vi "Create Single AO.vi"(7 "section":string, 8 "error in (no error)":errorcluster, 9 "AO_Channel":string(combo)="AO_Channel", 10 "Modbus_Master.lvclass":refnum<class "Modbus_Master.lvclass">, 11 "Config File In":path) -> (0 "error out":errorcluster, 2 "AnalogOutput.lvclass":refnum<class "AnalogOutput.lvclass">, 3 "Config File Out":path)   [LabVIEW 2021]
uses:
  AnalogOutput/AnalogOutput.lvclass
  Modbus_Master/Modbus_Master.lvclass
  Modbus_AO/Modbus_AO.lvclass
  C:/Users/lincoln.lucio/Documents/Lincoln/Documentos Pessoais/meus docs/Projetos pessoais/Projeto Sciranda/projeto_versioned/sciranda/AnalogOutput/AnalogOutput.lvclass
  Modbus_AO/Modbus_AO.lvclass/Modbus_AO.ctl
  DAQNavi_AO.lvclass/DAQNavi_AO.lvclass
  DAQNavi_AO.lvclass/DAQNavi_AO.lvclass/DAQNavi_AO.ctl
  Modbus_AO/Accessor VIs/Write Modbus_Master.lvclass.vi
  Modbus_AO/Accessor VIs/Write Register Address.vi
  Modbus_AO/Accessor VIs/Write Is Signed (I16)_.vi
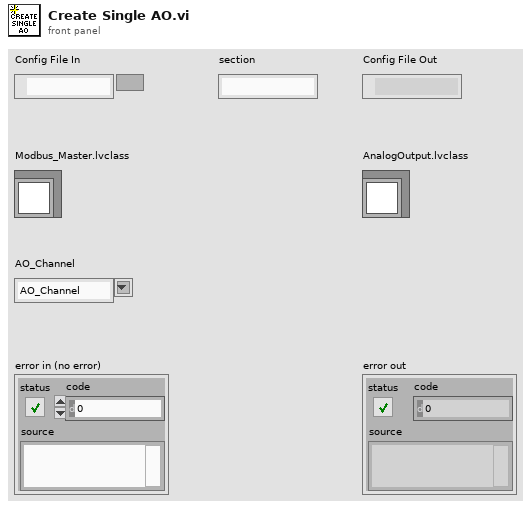
[diagram p1: front panel]
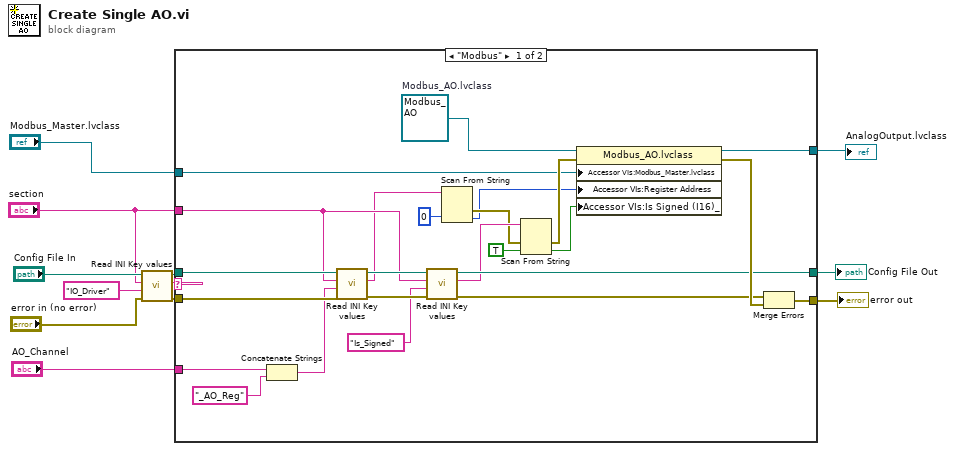
[diagram p0: block diagram]
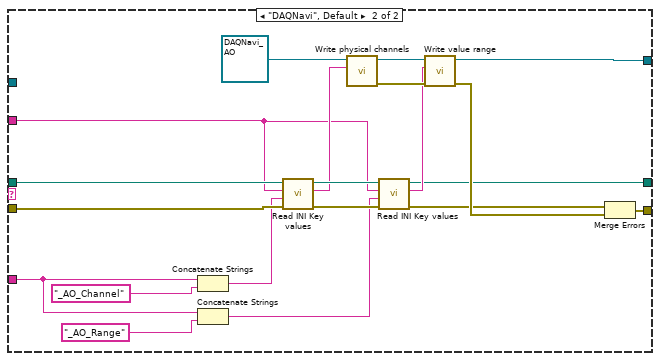
[diagram p2: hidden frame]
diagram:
  n1 = call "Read INI Key values.vi"("error in (no error)"="error in (no error)", "key"="IO_Driver", "section"="section", "Path In"="Config File In") -> ("error out"=w5:errorcluster, "value"=w9:string, "Path Out"=w7:path)  [unwired: 5 in]
  n2 = case shown="\"Modbus\"" w9 {
    tunnel: "AO_Channel" -> [w16 w40]
    tunnel: w7 -> [w32 w49]
    tunnel: w5 -> [w31 w48]
    tunnel: "section" -> [w28 w47]
    tunnel: [w25 w44] -> w11
    tunnel: [w34 w43] -> w10
    tunnel: [w35 w42] -> w3
    tunnel: "Modbus_Master.lvclass" -> [w13 _]
    frame "Modbus" {
      w36 = refnum<class "Modbus_AO.lvclass"> refnum  # Modbus_AO.lvclass
      n3 = Concatenate Strings(w16, "_AO_Reg" ("key")) -> (w14:string)
      n4 = call "Read INI Key values.vi"("error in (no error)"=w31, "key"=w14, "section"=w28, "Path In"=w32) -> ("error out"=w29:errorcluster, "value"=w17:string, "Path Out"=w30:path)  [unwired: 5 in]
      n5 = call "Read INI Key values.vi"("error in (no error)"=w29, "key"="Is_Signed", "section"=w28, "Path In"=w30) -> ("error out"=w26:errorcluster, "value"=w23:string, "Path Out"=w25:path)  [unwired: 5 in]
      n6 = Scan From String(input string=w17, default 1=u16 0 ("Register Address")) -> (error out=w19:errorcluster, output 1=w18:u16)  [unwired: 3 in, 2 out]
      n7 = Scan From String(input string=w23, error in=w19, default 1=TRUE ("Is Signed (I16)_")) -> (error out=w21:errorcluster, output 1=w22:bool)  [unwired: 2 in, 2 out]
      n8 = property class="Modbus_AO.lvclass"(reference=w36, error in=w21, "Accessor VIs:Modbus_Master.lvclass"=w13, "Accessor VIs:Register Address"=w18, "Accessor VIs:Is Signed (I16)_"=w22) -> (reference out=w35:refnum<class "Modbus_AO.lvclass">, error out=w33:errorcluster)
      n9 = Merge Errors(w26, w33) -> (w34:errorcluster)
    }
    frame "DAQNavi", Default {
      n10 = Concatenate Strings(w40, "_AO_Channel" ("string")) -> (w41:string)
      n11 = Concatenate Strings(w40, "_AO_Range" ("string")) -> (w37:string)
      n12 = call "Read INI Key values.vi"("error in (no error)"=w48, "key"=w41, "section"=w47, "Path In"=w49) -> ("error out"=w55:errorcluster, "value"=w54:string, "Path Out"=w56:path)  [unwired: 5 in]
      n13 = call "Write physical channels.vi"("physical channels"=w54, "DAQNavi_AO in"=refnum<class "DAQNavi_AO.lvclass"> refnum ("DAQNavi_AO.lvclass")) -> ("error out"=w52:errorcluster, "DAQNavi_AO out"=w51:refnum<class "DAQNavi_AO.lvclass">)  [unwired: 8 in]
      n14 = call "Read INI Key values.vi"("error in (no error)"=w55, "key"=w37, "section"=w47, "Path In"=w56) -> ("error out"=w45:errorcluster, "value"=w50:string, "Path Out"=w44:path)  [unwired: 5 in]
      n15 = call "Write value range.vi"("error in (no error)"=w52, "value range"=w50, "DAQNavi_AO in"=w51) -> ("error out"=w46:errorcluster, "DAQNavi_AO out"=w42:refnum<class "DAQNavi_AO.lvclass">)  [unwired: 7 in]
      n16 = Merge Errors(w45, w46) -> (w43:errorcluster)
    }
  }
  "Config File Out" <- w11
  "error out" <- w10
  "AnalogOutput.lvclass" <- w3
